vi "Mise a jour liste Selection.vi"(7 "RéfCmde sélection":refnum<vi>, 8 "error in (no error)":errorcluster, 11 "Choisir capteur parmis":refnum<vi>) -> (0 "error out":errorcluster, 3 "Capteurs choisit":string[](array[string]))   [LabVIEW 2022 SP3]
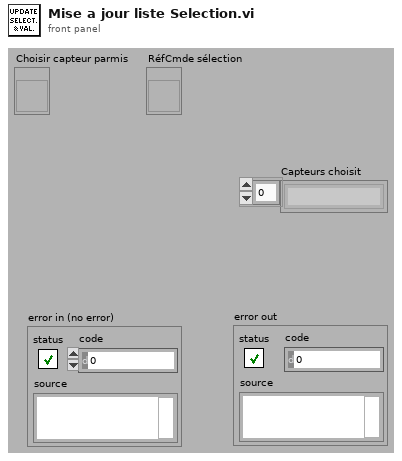
[diagram p1: front panel]
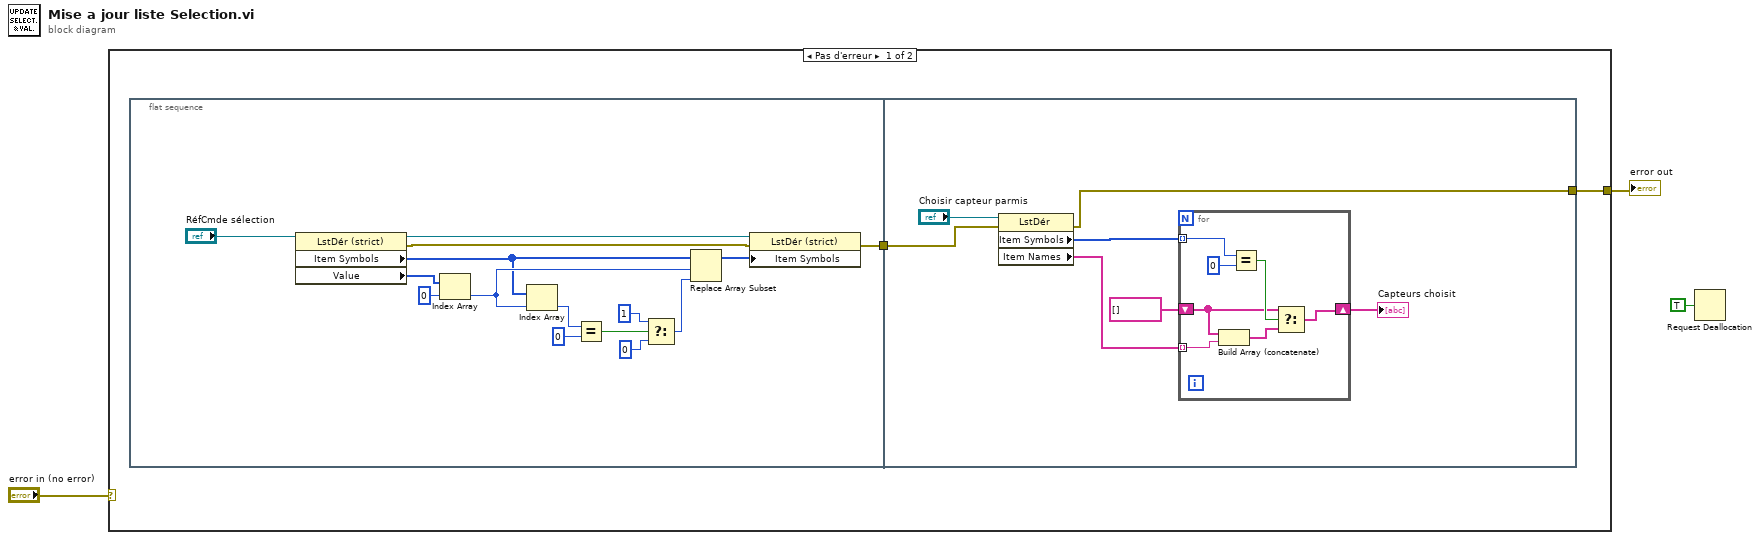
[diagram p0: block diagram]
diagram:
  n1 = case shown="Pas d'erreur" "error in (no error)" {
    selector: "error in (no error)" -> [_ w35]
    tunnel: [w4 w35] -> w2
    frame No Error {
      n2 = flat-sequence {
        tunnel: [w6] -> w5
        tunnel: w5 -> [w22]
        tunnel: [w21] -> w4
        frame #0 {
          n3 = property class="LstDér (strict)"(reference="RéfCmde sélection") -> (reference out=w9:refnum<vi>, error out=w7:errorcluster, "Item Symbols"=w8:i32[], "Value"=w12:i32[])  [unwired: 1 in]
          n4 = Index Array(array=w12, index=0 ("indice")) -> (element=w10:i32)
          n5 = Index Array(array=w8, index=w10) -> (element=w15:i32)
          n6 = Equal?(x=w15, y=0) -> (x = y?=w17:bool)
          n7 = Select(t=1 ("y"), s=w17, f=0 ("y")) -> (s? t:f=w18:i32)
          n8 = Replace Array Subset(array=w8, new element=w18, index=w10) -> (w14:i32[])
          n9 = property on="Property Node" class="LstDér (strict)"(reference=w9, error in=w7, "Item Symbols"=w14) -> (error out=w6:errorcluster)  [unwired: 1 out]
        }
        frame #1 {
          n10 = property on="Property Node" class="LstDér"(reference="Choisir capteur parmis", error in=w22) -> (error out=w21:errorcluster, "Item Symbols"=w25:i32[], "Item Names"=w27:string[])  [unwired: 1 out]
          n11 = for {
            tunnel: w27 -> [w31] mode=indexing
            tunnel: w25 -> [w33] mode=indexing
            shift-right: [w30] -> w23
            shift-left: string[] [] -> [w29]
            n12 = Build Array (concatenate)(w29, w31) -> (w28:string[])
            n13 = Equal?(x=w33, y=0) -> (x = y?=w32:bool)
            n14 = Select(t=w29, s=w32, f=w28) -> (s? t:f=w30:string[])
          }
          "Capteurs choisit" <- w23
        }
      }
    }
    frame Error {
    }
  }
  "error out" <- w2
  n15 = Request Deallocation(TRUE ("flag")) -> ()
